vi "Smart IO Get Analog Voltage.vi"(6 "force":bool, 8 "error in (no error)":errorcluster, 11 "deviceIndex":i32=-1) -> (0 "error out":errorcluster, 1 "Raw Value":u32, 2 "Volts":dbl)   [LabVIEW 2023, in "MrcLib.lvlib"]
doc: "Returns the voltage value directly from the A/D converter on the channel. The converter scales the raw value to the voltage value using the least significant bit weight constant and the offset constant of the hardware. If changing I/O types, you can force the channel type."
uses:
  <vilib>/MRC/MrcLib.lvlib
  <vilib>/MRC/Types/MRC Smart IO Mode.ctl
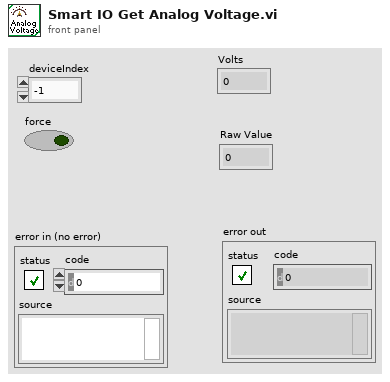
[diagram p1: front panel]
types:
  T1 = typedef "MRC Smart IO Mode.ctl" = i32
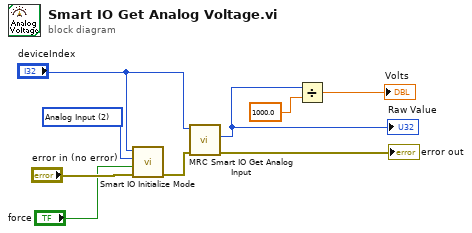
[diagram p0: block diagram]
diagram:
  w5 = T1 2 items=["Digital Input"=0, "Digital Output"=1, "Analog Input"=2, "PWM Input"=3, "PWM Output"=4, "Counter Rising"=5, "Counter Falling"=6, "Addressable LEDs"=13] ("mode")
  n1 = call <vilib>:"Smart IO Initialize Mode.vi"("error in (no error)"="error in (no error)", "force"="force", "mode"=w5, "deviceIndex"="deviceIndex") -> ("error out"=w7:errorcluster)  [unwired: 7 in]
  n2 = call <vilib>:"MRC Smart IO Get Analog Input.vi"("error in (no error)"=w7, "deviceIndex"="deviceIndex") -> ("error out"=→"error out":errorcluster, "value out"=w2:i32)  [unwired: 8 in]
  "Raw Value" <- w2
  n3 = Divide(x=w2, y=1000.0) -> (x/y=→"Volts":dbl)
